vi "calculate_strain_from_array__a6961fd85f.vi"(7 "real strain":dbl[](array[numeric]), 9 "Gap":dbl, 10 "voltage to displacement contant":dbl) -> (2 "real strain (-)":dbl[](array[numeric]))   [LabVIEW 2023]
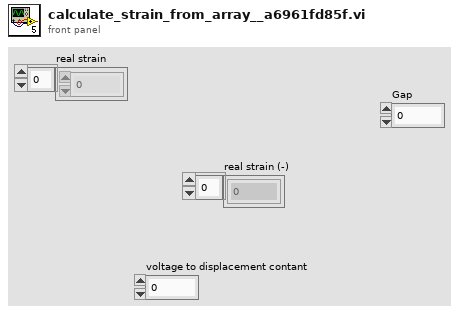
[diagram p1: front panel]
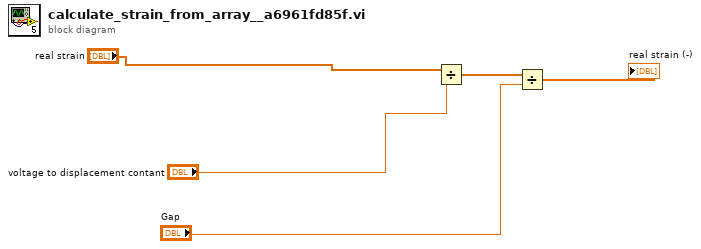
[diagram p0: block diagram]
diagram:
  n1 = Divide(x="real strain", y="voltage to displacement contant") -> (x/y=w4:dbl[])
  n2 = Divide(x=w4, y="Gap") -> (x/y=→"real strain (-)":dbl[])
